vi "Dispatch Probe 2.vi"() -> (0 "answer":string)   [LabVIEW 2026]
doc: "Round15 P15 v2: the type-launderer chain. seed (class constant) feeds Sensor:Scale By, whose obj out is a SENSOR-typed wire; that wire feeds Sensor:Tag. Because Tag's input arrives parent-typed, the editor cannot bind it at edit time, so the runtime value (a Temp Sensor) must select the implementation - dynamic dispatch, observed. answer=Temp Sensor with both calls still on Sensor members proves it."
uses:
  lib/Temp Sensor.lvclass
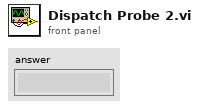
[diagram p1: front panel]
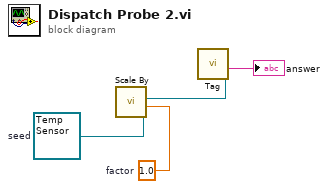
[diagram p0: block diagram]
diagram:
  w2 = 1.0  # factor
  w1 = refnum<class "Temp Sensor.lvclass"> refnum  # seed
  n1 = call-dynamic "Scale By.vi"("obj in"=w1, "Factor"=w2) -> ("obj out"=w4:refnum<class "Temp Sensor.lvclass">)  [unwired: 9 in]
  n2 = call-dynamic "Tag.vi"("obj in"=w4) -> ("tag"=→"answer":string)  [unwired: 10 in]
